vi "Get Tx Configuration.vi"(8 "error in":errorcluster, 11 "custom device":T1 format="%.0x") -> (0 "error out":errorcluster, 2 "configuration string out":string, 3 "custom device out":T1 format="%.0x")   [LabVIEW 2020, in "Ballard ARINC 429 Hardware Configuration.lvlib"]
uses:
  Ballard ARINC 429 Hardware Configuration.lvlib
  <vilib>/NI VeriStand/Custom Device API/Custom Device Item Ref.ctl
  Constants.vi
  Scripting/Ballard/Ballard ARINC 429 Scripting.lvlib
  Scripting/ARINC 429/ARINC 429 Scripting.lvlib
  <vilib>/NI VeriStand/Custom Device API/Custom Device API.lvlib
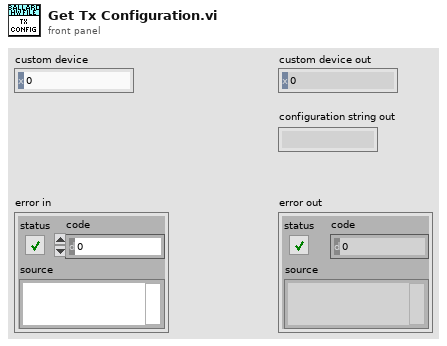
[diagram p1: front panel]
types:
  T1 = typedef "Custom Device API.lvlib/Custom Device Item Ref.ctl" = u64
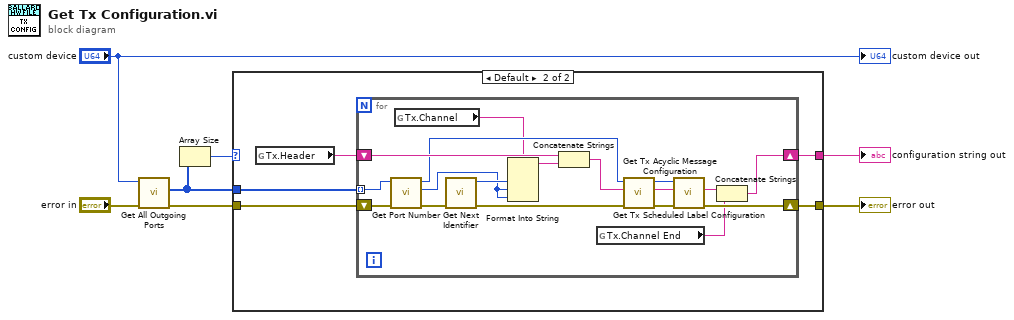
[diagram p0: block diagram]
diagram:
  n1 = call "Get All Outgoing Ports.vi"("error in"="error in", "Ballard ARINC 429 custom device in"="custom device") -> ("error out"=w5:errorcluster, "outgoing ports"=w2:T1[])  [unwired: 7 in, 1 out]
  n2 = Array Size(array=w2) -> (size(s)=w1:i32)
  n3 = case shown="Default" w1 {
    tunnel: w2 -> [_ w13]
    tunnel: [w8 w12] -> w7
    tunnel: w5 -> [w8 w11]
    tunnel: [_ w10] -> w4
    frame ..0 {
    }
    frame Default {
      n4 = global read "Constants.vi" "Tx.Header"() -> (w9:string)
      n5 = for {
        tunnel: w13 -> [w31] mode=indexing
        shift-right: [w23] -> w10
        shift-left: w9 -> [w27]
        shift-right: [w25] -> w12
        shift-left: w11 -> [w30]
        n6 = call "Get Port Number.vi"("error in"=w30, "port ref in"=w31) -> ("error out"=w29:errorcluster, "port number"=w16:u16, "port ref out"=w21:T1)  [unwired: 6 in, 1 out]
        n7 = global read "Constants.vi" "Tx.Channel"() -> (w15:string)
        n8 = call "Get Next Identifier.vi"("error in"=w29) -> ("error out"=w18:errorcluster, "ID"=w28:u32)  [unwired: 9 in]
        n9 = Format Into String(format string=w15, w28, w16, w16) -> (resulting string=w26:string)  [unwired: 2 in, 1 out]
        n10 = Concatenate Strings(w27, w26) -> (w22:string)
        n11 = global read "Constants.vi" "Tx.Channel End"() -> (w14:string)
        n12 = call "Get Tx Acyclic Message Configuration.vi"("error in"=w18, "configuration string"=w22, "port"=w21) -> ("error out"=w17:errorcluster, "configuration string out"=w20:string, "port out"=w19:T1)  [unwired: 6 in]
        n13 = call "Get Tx Scheduled Label Configuration.vi"("error in"=w17, "configuration string"=w20, "port"=w19) -> ("error out"=w25:errorcluster, "configuration string out"=w24:string)  [unwired: 6 in, 1 out]
        n14 = Concatenate Strings(w24, w14) -> (w23:string)
      }
    }
  }
  "error out" <- w7
  "configuration string out" <- w4
  "custom device out" <- "custom device"
